vi "Timer_Start.vi"(8 "Pass_Through_Time":dbl=-1.0 format="%33.4f", 11 "in Timer":T1 {"Accumulated TIme" format="%13.5p"; "StartTime" format="%13.5p"}) -> (3 "out Timer":T1 {"Accumulated TIme" format="%13.5p"; "StartTime" format="%13.5p"})   [LabVIEW 2019, in "Trajectory_Library.lvlib"]
doc: "Start the timer running. Just set the running flag to true indicating that all time requests should be relative to the system clock.\n\nInputs:\n - Timer -- The Timer data cluster\n\nOutputs:\n - Timer -- The modified Timer data cluster"
uses:
  Trajectory_Library.lvlib
  TypeDef/TIMER.ctl
  VI/Util_GetTime_U32.vi
  VI/Util_GetTime_U64.vi
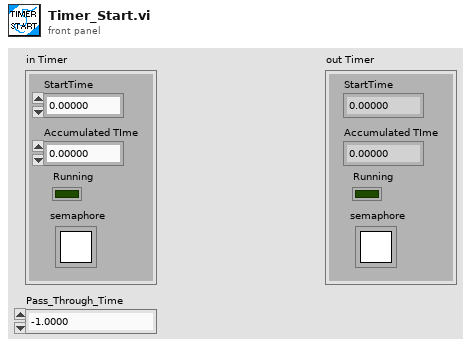
[diagram p1: front panel]
types:
  T1 = typedef "Trajectory_Library.lvlib/TIMER.ctl" = cluster{"StartTime":dbl, "Accumulated TIme":dbl, "Running":bool, "semaphore":T2}
  T2 = typedef "Semaphore RefNum" = refnum<k1>
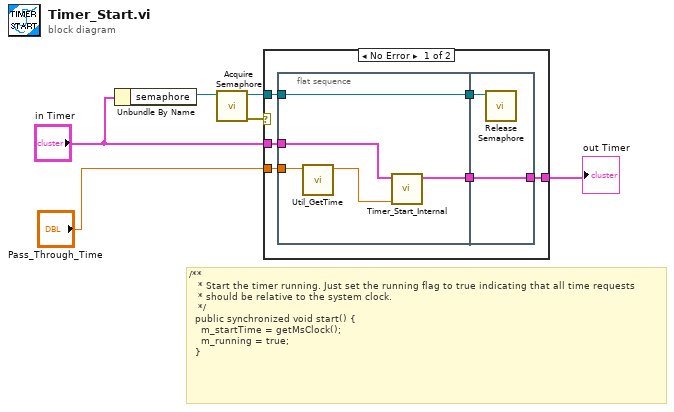
[diagram p0: block diagram]
diagram:
  # "/**\n   * Start the timer running. Just set the running flag to true indicating that all time requests\n   * should be relative to the system clock.\n   */\n  public synchronized void start() {\n    m_startTime = getMsClock();\n    m_running = true;\n  }"
  n1 = Unbundle By Name("in Timer") -> ("semaphore"=w5:T2)
  n2 = call <vilib>:"Acquire Semaphore.vi"("semaphore"=w5) -> ("error out"=w3:errorcluster, "semaphore out"=w2:T2)  [unwired: 4 in, 1 out]
  n3 = case shown="No Error" w3 {
    tunnel: "in Timer" -> [w12 w20]
    tunnel: [w11 w20] -> w6
    tunnel: w2 -> [w8 _]
    tunnel: "Pass_Through_Time" -> [w7 _]
    frame No Error {
      n4 = flat-sequence {
        tunnel: w12 -> [w17]
        tunnel: [w16] -> w10
        tunnel: [w15] -> w9
        tunnel: w8 -> [w15]
        tunnel: w7 -> [w14]
        tunnel: [w19] -> w11
        tunnel: w10 -> [w19]
        tunnel: w9 -> [w18]
        frame #0 {
          n5 = call "Util_GetTime.vi"("Pass_Through_Time"=w14) -> ("FPGA_Time_Seconds"=w13:dbl)  [unwired: 8 in, 2 out]
          n6 = call "Timer_Start_Internal.vi"("FPGA_Time_Seconds"=w13, "in Timer in"=w17) -> ("in Timer out"=w16:T1)  [unwired: 9 in]
        }
        frame #1 {
          n7 = call <vilib>:"Release Semaphore.vi"("semaphore"=w18) -> ()  [unwired: 5 in, 2 out]
        }
      }
    }
    frame Error {
    }
  }
  "out Timer" <- w6
